vi "CursorDraw.vi"(8 "error in (no error)":errorcluster, 9 "Coords":T1, 11 "Gviewer in":refnum<class "Gviewer.lvclass">) -> (0 "error out":errorcluster, 3 "Gviewer out":refnum<class "Gviewer.lvclass">)   [LabVIEW 2020, in "Sgraph_lib_V1.lvlib" / "Gviewer.lvclass"]
doc: "Draw info at cursor point"
uses:
  Gviewer.lvclass
  <vilib>/Utility/miscctls.llb/LVPoint32TypeDef.ctl
  Gviewer.lvclass/Gviewer.ctl
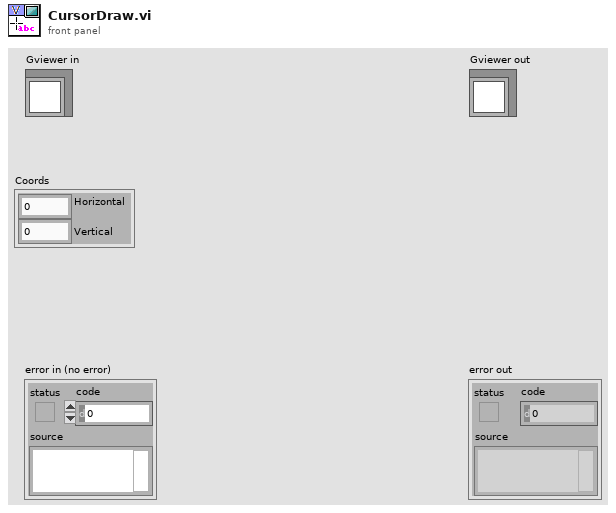
[diagram p1: front panel]
types:
  T1 = typedef "LVPoint32TypeDef.ctl" = cluster{"Horizontal":i32, "Vertical":i32}
  T2 = cluster{"horizontal":enum16{"left", "center", "right"}, "vertical":enum16{"top", "center", "bottom"}}
  T3 = typedef "LVRectTypeDef.ctl" = cluster{"Left":i16, "Top":i16, "Right":i16, "Bottom":i16}
  T4 = typedef "Sgraph_lib_V1.lvlib/Gviewer.lvclass/Typedef_Live.ctl" = enum16{"Live View", "Freeze"}
  T5 = typedef "Sgraph_lib_V1.lvlib/FAMM.lvclass/FAMM_reply_datagram.ctl" = cluster{"GraphName":string, "Time-Start":timestamp, "Time-End":timestamp, "TimeSpan":dbl, "Live":T4, "WAQ_section":T6, "EAQ_section":T7, "PAQ_section":T8, "Layer":i32}
  T6 = typedef "Sgraph_lib_V1.lvlib/FAMM.lvclass/FAMM_reply_WAQdata.ctl" = cluster{"Boolean":bool}
  T7 = typedef "Sgraph_lib_V1.lvlib/FAMM.lvclass/FAMM_reply_EAQdata.ctl" = cluster{"Boolean":bool}
  T8 = typedef "Sgraph_lib_V1.lvlib/FAMM.lvclass/FAMM_reply_PAQdata.ctl" = cluster{"Tags":string[], "time stamp":timestamp[], "DataSection":cluster{"data":dbl[], "max":dbl[], "min":dbl[], "Status":u32[]}[]}
  T9 = typedef "Sgraph_lib_V1.lvlib/Gviewer.lvclass/LegendSet.ctl" = cluster{"Position":T10, "Size":T11, "Rows":u32, "Select":i32, "Visible":bool}
  T10 = typedef "LVPositionTypeDef.ctl" = cluster{"Left":i32, "Top":i32}
  T11 = typedef "LVBoundsTypeDef.ctl" = cluster{"Width":u32, "Height":u32}
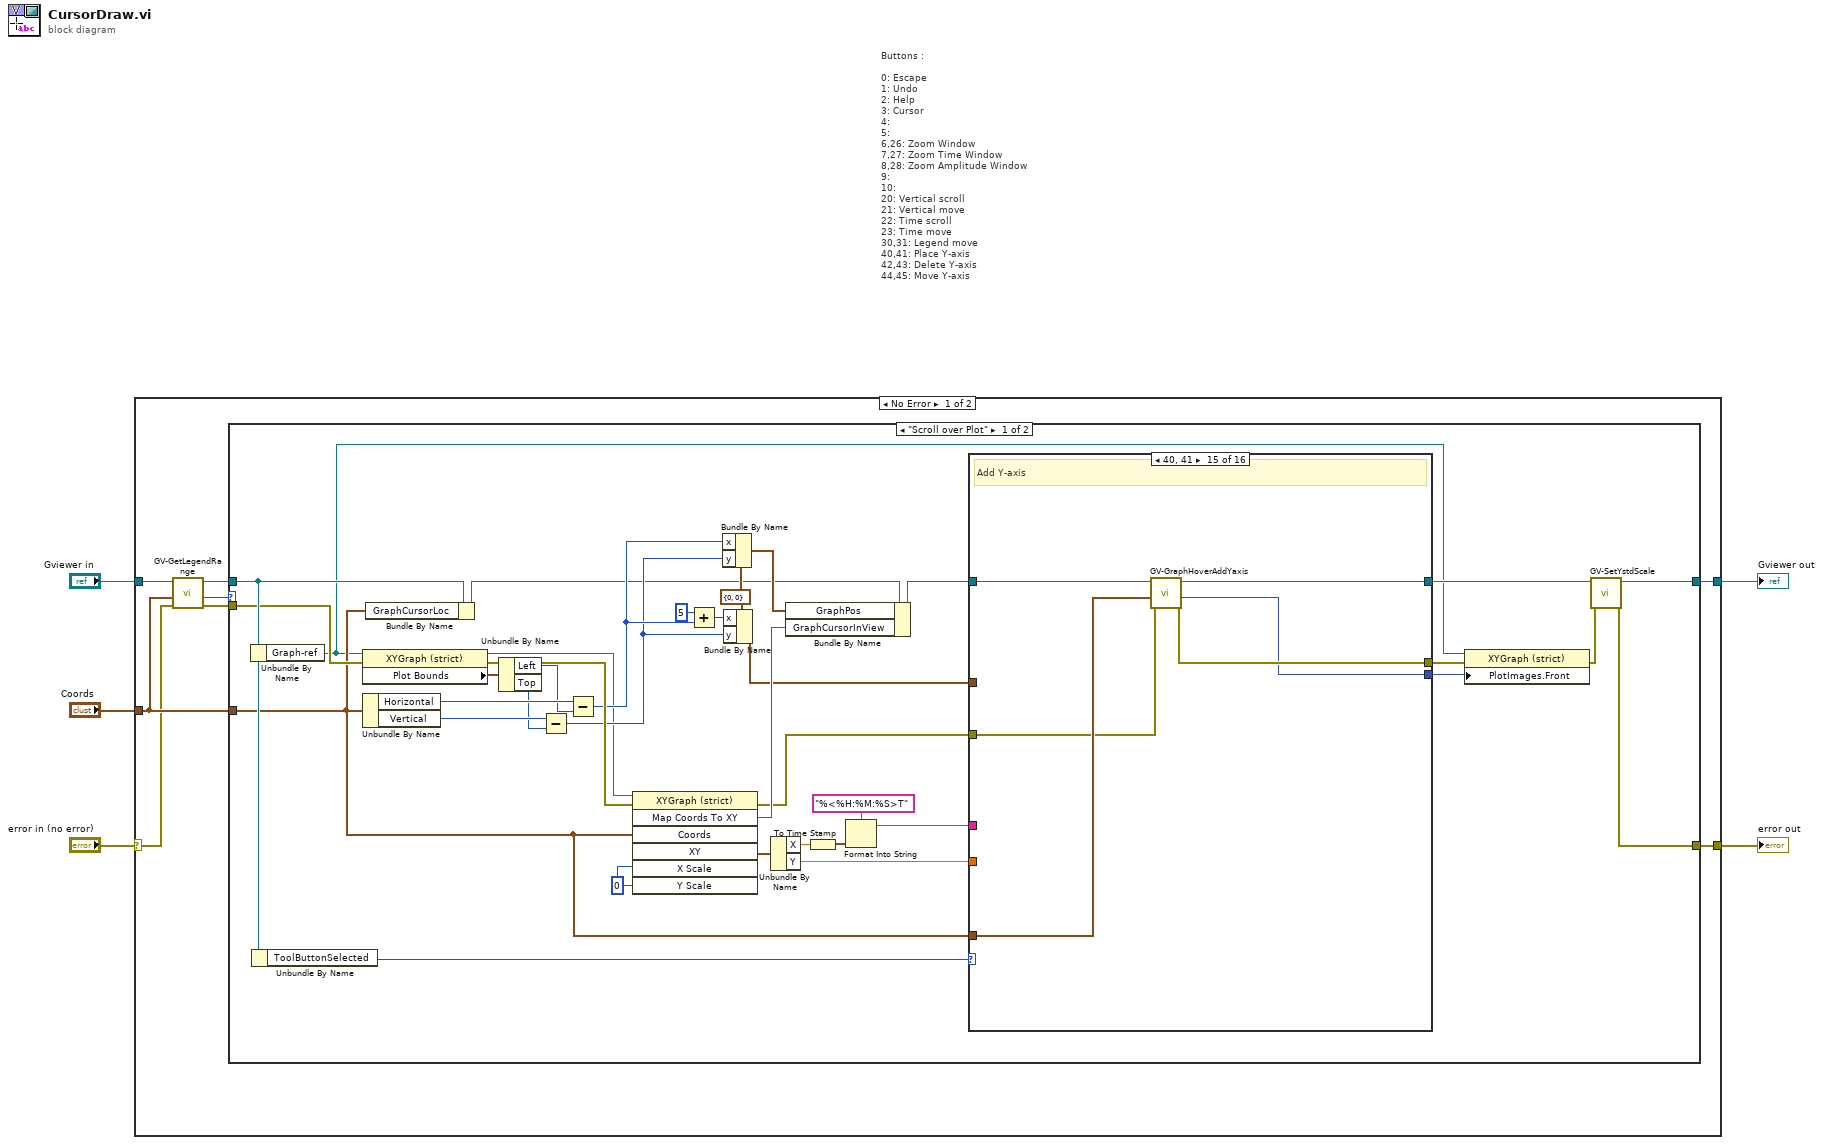
[diagram p0: block diagram]
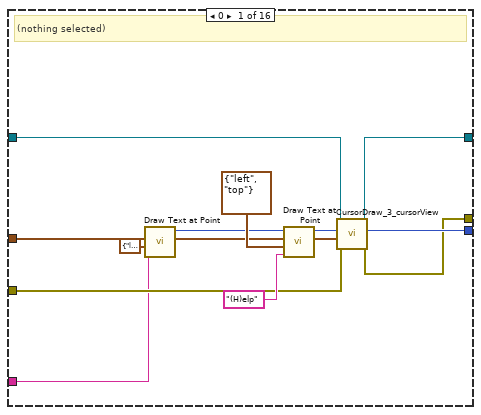
[diagram p2: hidden frame]
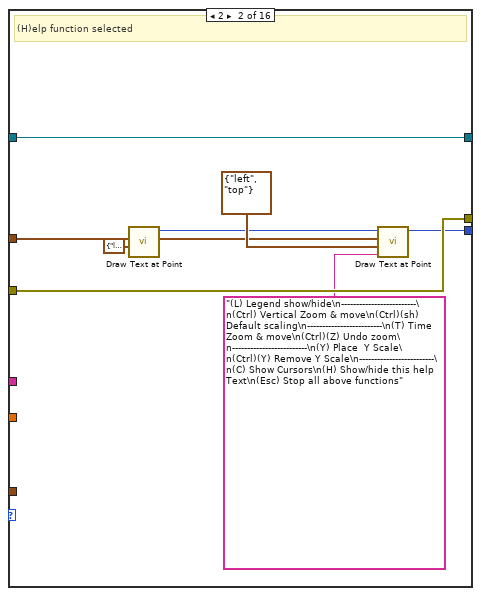
[diagram p3: hidden frame]
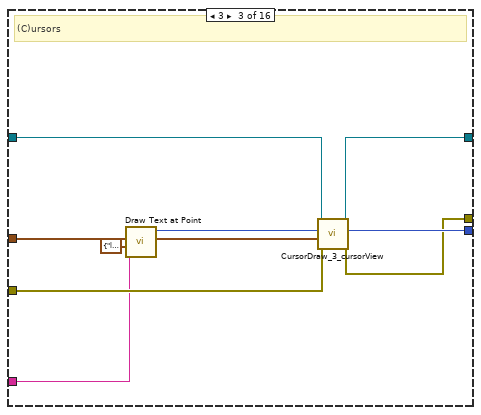
[diagram p4: hidden frame]
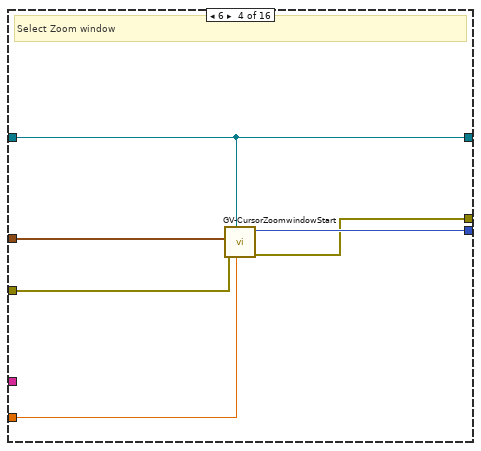
[diagram p5: hidden frame]
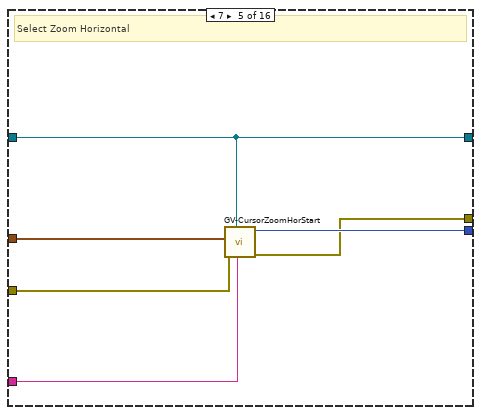
[diagram p6: hidden frame]
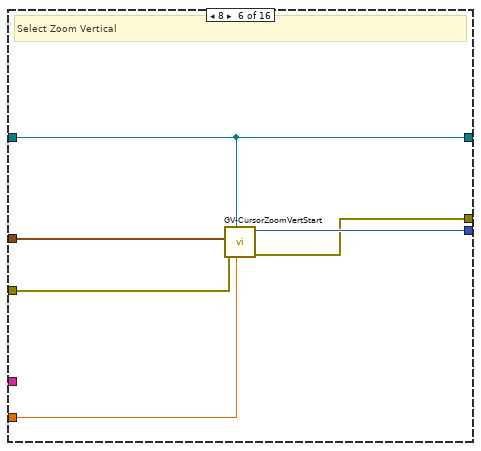
[diagram p7: hidden frame]
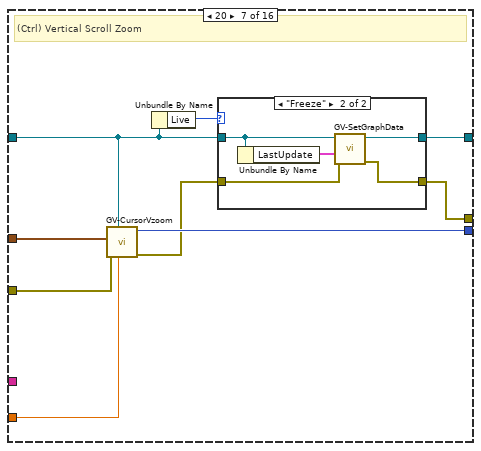
[diagram p8: hidden frame]
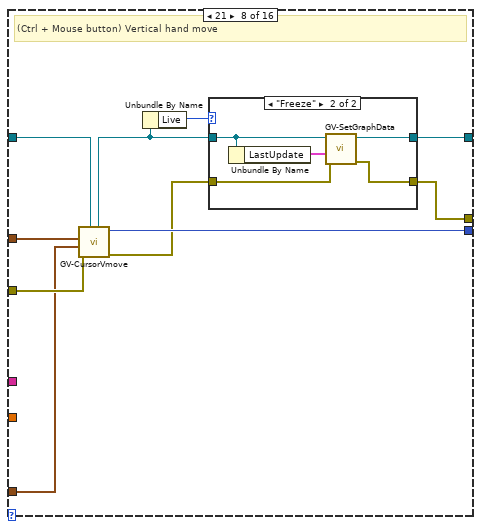
[diagram p10: hidden frame]
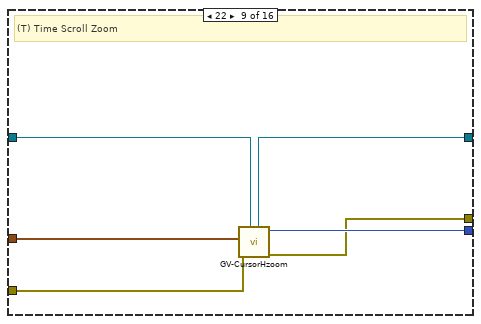
[diagram p12: hidden frame]
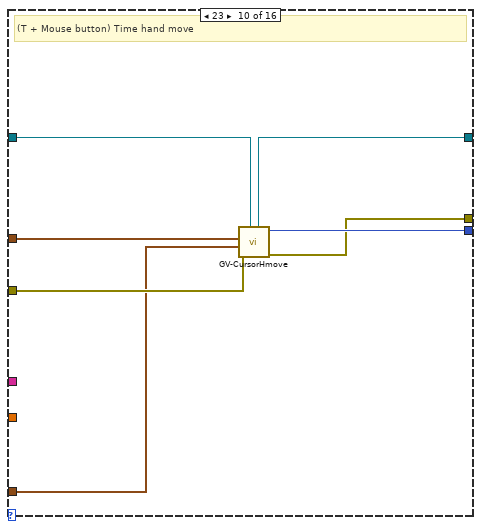
[diagram p13: hidden frame]
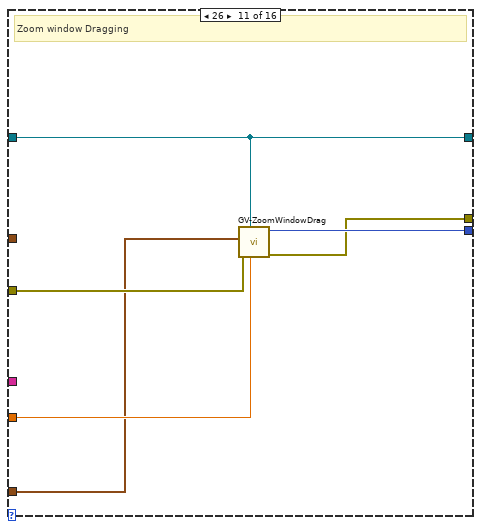
[diagram p14: hidden frame]
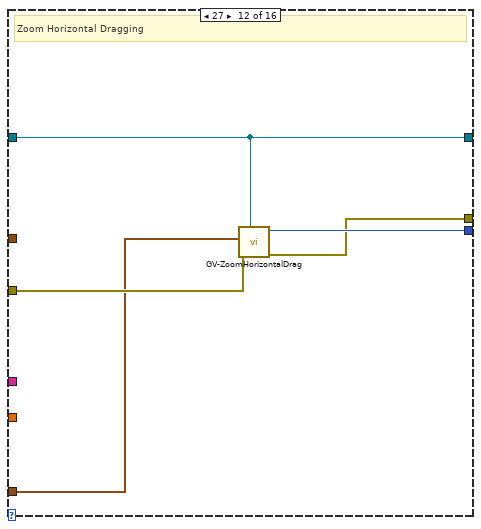
[diagram p15: hidden frame]
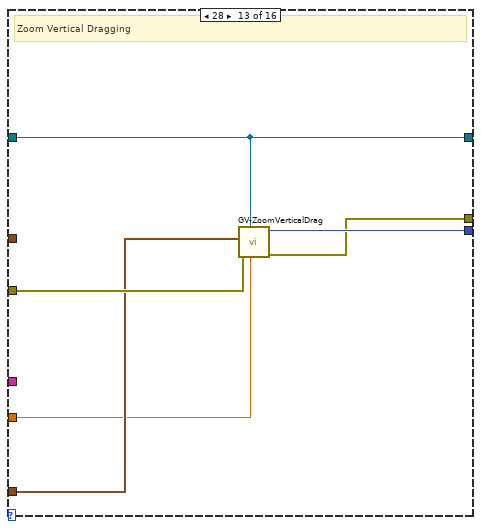
[diagram p16: hidden frame]
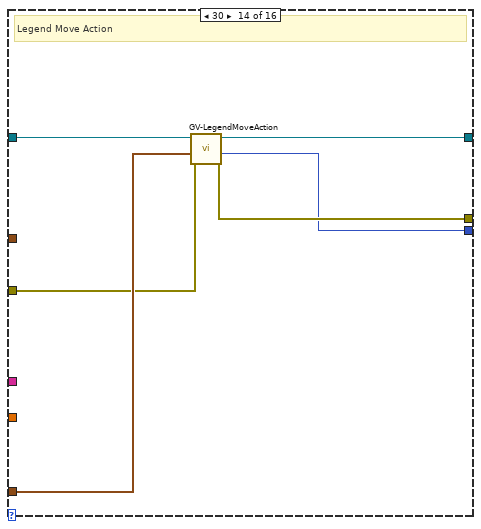
[diagram p17: hidden frame]
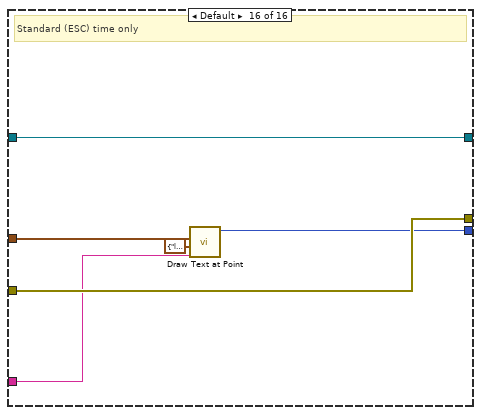
[diagram p18: hidden frame]
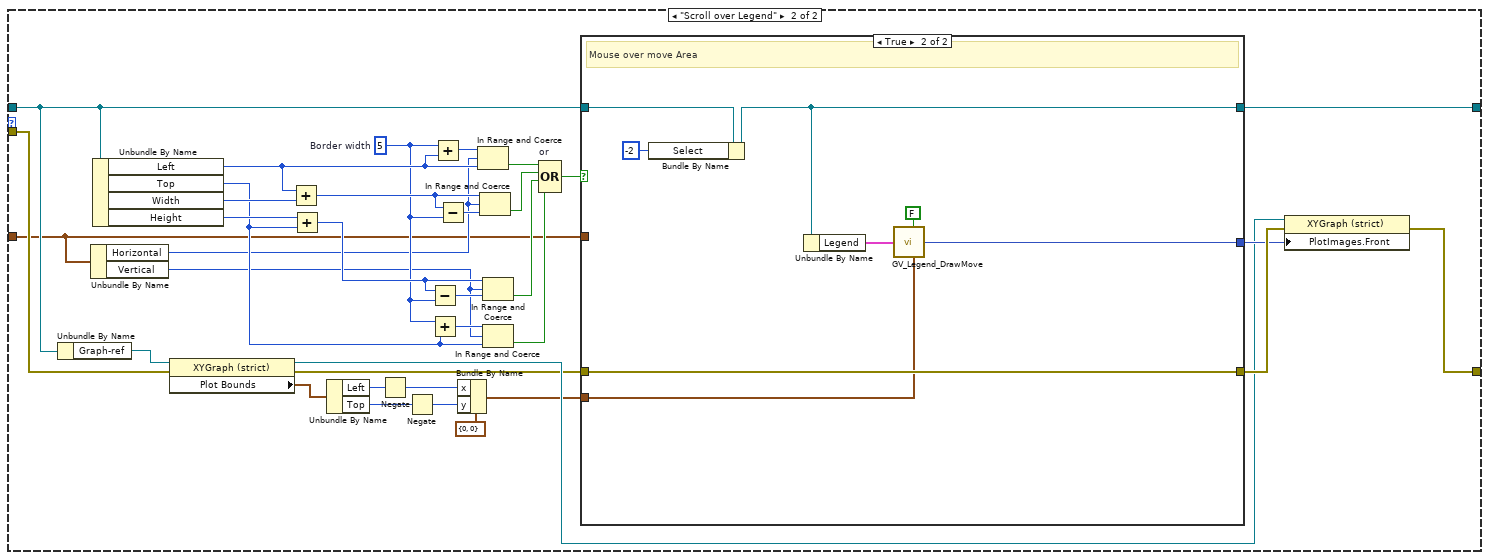
[diagram p19: hidden frame]
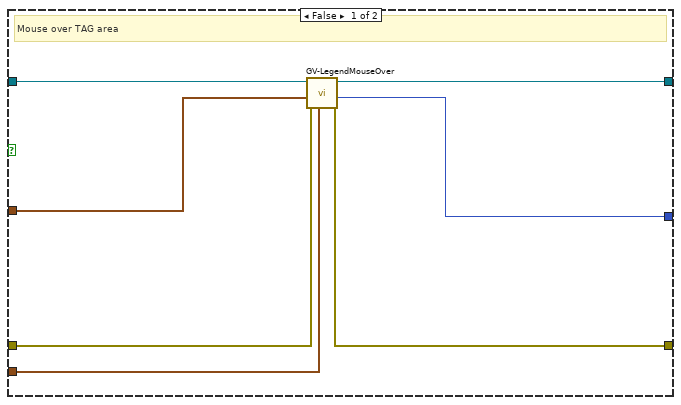
[diagram p20: hidden frame]
diagram:
  # "Buttons :\n\n0: Escape\n1: Undo\n2: Help\n3: Cursor\n4: \n5:\n6,26: Zoom Window\n7,27: Zoom Time Window\n8,28: Zoom Amplitude Window\n9:\n10:\n20: Vertical scroll\n21: Vertical move\n22: Time scroll\n23: Time move\n30,31: Legend move\n40,41: Place Y-axis\n42,43: Delete Y-axis\n44,45: Move Y-axis"
  n1 = case shown="No Error" "error in (no error)" {
    selector: "error in (no error)" -> [w6 w229]
    tunnel: [w12 w229] -> w4
    tunnel: [w13 w228] -> w2
    tunnel: "Gviewer in" -> [w10 w228]
    tunnel: "Coords" -> [w8 _]
    frame No Error {
      n2 = call "GV-GetLegendRange.vi"("error in (no error)"=w6, "Coords"=w8, "Gviewer in"=w10) -> ("error out"=w9:errorcluster, "Where?"=w7:enum16{"Scroll over Plot", "Scroll over Legend"}, "Gviewer out"=w11:refnum<class "Gviewer.lvclass">)  [unwired: 6 in]
      n3 = case shown="\"Scroll over Plot\"" w7 {
        tunnel: [w22 w178] -> w13
        tunnel: [w20 w179] -> w12
        tunnel: w11 -> [w19 w196]
        tunnel: w9 -> [w18 w181]
        tunnel: w8 -> [w17 w180]
        frame "Scroll over Plot" {
          w43 = 0 ("Y Scale")
          w31 = cluster{"x":i16, "y":i16} {"x"=0, "y"=0} ("origin")
          n4 = Unbundle By Name(w19) -> ("Graph-ref"=w14:refnum<vi>)
          n5 = Unbundle By Name(w19) -> ("ToolButtonSelected"=w26:i32)
          n6 = property class="XYGraph (strict)"(reference=w14, error in=w18) -> (reference out=w15:refnum<vi>, error out=w44:errorcluster, "Plot Bounds"=w49:T3)
          n7 = Unbundle By Name(w17) -> ("Horizontal"=w48:i32, "Vertical"=w47:i32)
          n8 = Bundle By Name(cluster=w19, "GraphCursorLoc"=w17) -> (w27:refnum<class "Gviewer.lvclass">)
          n9 = Unbundle By Name(w49) -> ("Left"=w46:i16, "Top"=w45:i16)
          n10 = Subtract(x=w47, y=w45) -> (x-y=w29:i32)
          n11 = Subtract(x=w48, y=w46) -> (x-y=w30:i32)
          n12 = invoke class="XYGraph (strict)" method="Map Coords To XY"(reference=w15, error in=w44, "Coords"=w17, "X Scale"=w43, "Y Scale"=w43) -> (error out=w33:errorcluster, "Map Coords To XY"=w41:bool, "XY"=w42:cluster{"X":dbl, "Y":dbl})  [unwired: 2 in, 4 out]
          n13 = Add(x=5, y=w30) -> (x+y=w36:i32)
          n14 = Bundle By Name(cluster=w31, "x"=w30, "y"=w29) -> (w28:cluster{"x":i16, "y":i16})
          n15 = Bundle By Name(cluster=w31, "x"=w36, "y"=w29) -> (w24:cluster{"x":i16, "y":i16})
          n16 = Unbundle By Name(w42) -> ("X"=w40:dbl, "Y"=w23:dbl)
          n17 = Bundle By Name(cluster=w27, "GraphPos"=w28, "GraphCursorInView"=w41) -> (w35:refnum<class "Gviewer.lvclass">)
          n18 = To Time Stamp(1:w40) -> (0:w39:timestamp)
          n19 = Format Into String(format string="%<%H:%M:%S>T", w39) -> (resulting string=w25:string)  [unwired: 2 in, 1 out]
          n20 = case shown="40, 41" w26 {
            tunnel: w35 -> [w56 w69 w77 w80 w86 w92 w98 w120 w130 w136 w145 w150 w156 w165 w171 w177]
            tunnel: [w58 w67 w76 w84 w90 w96 w105 w118 w135 w142 w148 w153 w159 w160 w166 w174] -> w34
            tunnel: [w57 w69 w78 w80 w86 w92 w101 w115 w131 w137 w145 w150 w156 w163 w169 w177] -> w16
            tunnel: w33 -> [w54 w68 w74 w83 w89 w95 w104 w122 w133 w140 w146 w151 w157 w162 w168 w176]
            tunnel: [w55 w68 w75 w82 w88 w94 w99 w113 w134 w141 w147 w152 w158 w161 w167 w176] -> w32
            tunnel: w25 -> [w50 _ w70 _ w85 _ _ _ _ _ _ _ _ _ _ w173]
            tunnel: w24 -> [w51 w62 w72 w81 w87 w93 w103 w119 w132 w139 _ _ _ _ _ w172]
            tunnel: w23 -> [_ _ _ w79 _ w91 w102 _ _ _ w144 _ w154 _ _ _]
            tunnel: w17 -> [_ _ _ _ _ _ _ w121 _ w138 w143 w149 w155 w164 w170 _]
            frame 0 {
              # "(nothing selected)"
              n21 = call <vilib>:"Draw Text at Point.vi"("text"=w50, "alignment(left, top)"=T2 {"horizontal"=enum."left", "vertical"=enum."bottom"}, "origin"=w51) -> ("new picture"=w52:picture)  [unwired: 7 in, 1 out]
              n22 = call <vilib>:"Draw Text at Point.vi"("text"="(H)elp", "alignment(left, top)"=T2 {"horizontal"=enum."left", "vertical"=enum."top"}, "origin"=w51, "picture"=w52) -> ("new picture"=w59:picture)  [unwired: 6 in, 1 out]
              n23 = call "CursorDraw_3_cursorView.vi"("error in (no error)"=w54, "Pos"=w51, "pict in"=w59, "Gviewer in"=w56) -> ("error out"=w55:errorcluster, "pict out"=w58:picture, "Gviewer out"=w57:refnum<class "Gviewer.lvclass">)  [unwired: 5 in]
            }
            frame 2 {
              # "(H)elp function selected"
              n24 = call <vilib>:"Draw Text at Point.vi"("alignment(left, top)"=T2 {"horizontal"=enum."left", "vertical"=enum."bottom"}, "origin"=w62) -> ("new picture"=w63:picture)  [unwired: 8 in, 1 out]
              n25 = call <vilib>:"Draw Text at Point.vi"("text"="(L) Legend show/hide\n-------------------------\n(Ctrl) Vertical Zoom & move\n(Ctrl)(sh) Default scaling\n-------------------------\n(T) Time Zoom & move\n(Ctrl)(Z) Undo zoom\n-------------------------\n(Y) Place  Y Scale\n(Ctrl)(Y) Remove Y Scale\n-------------------------\n(C) Show Cursors\n(H) Show/hide this help Text\n(Esc) Stop all above functions", "alignment(left, top)"=T2 {"horizontal"=enum."left", "vertical"=enum."top"}, "origin"=w62, "picture"=w63) -> ("new picture"=w67:picture)  [unwired: 6 in, 1 out]
            }
            frame 3 {
              # "(C)ursors"
              n26 = call <vilib>:"Draw Text at Point.vi"("text"=w70, "alignment(left, top)"=T2 {"horizontal"=enum."left", "vertical"=enum."bottom"}, "origin"=w72) -> ("new picture"=w71:picture)  [unwired: 7 in, 1 out]
              n27 = call "CursorDraw_3_cursorView.vi"("error in (no error)"=w74, "Pos"=w72, "pict in"=w71, "Gviewer in"=w77) -> ("error out"=w75:errorcluster, "pict out"=w76:picture, "Gviewer out"=w78:refnum<class "Gviewer.lvclass">)  [unwired: 5 in]
            }
            frame 6 {
              # "Select Zoom window"
              n28 = call "GV-CursorZoomwindowStart.vi"("Y"=w79, "Gviewer in"=w80, "error in (no error)"=w83, "Pos"=w81) -> ("error out"=w82:errorcluster, "pict out"=w84:picture)  [unwired: 6 in]
            }
            frame 7 {
              # "Select Zoom Horizontal"
              n29 = call "GV-CursorZoomHorStart.vi"("time"=w85, "Gviewer in"=w86, "error in (no error)"=w89, "Pos"=w87) -> ("error out"=w88:errorcluster, "pict out"=w90:picture)  [unwired: 6 in]
            }
            frame 8 {
              # "Select Zoom Vertical"
              n30 = call "GV-CursorZoomVertStart.vi"("Y"=w91, "Gviewer in"=w92, "error in (no error)"=w95, "Pos"=w93) -> ("error out"=w94:errorcluster, "pict out"=w96:picture)  [unwired: 6 in]
            }
            frame 20 {
              # "(Ctrl) Vertical Scroll Zoom"
              n31 = call "GV-CursorVzoom.vi"("Y"=w102, "Gviewer in"=w98, "error in (no error)"=w104, "Pos"=w103) -> ("error out"=w100:errorcluster, "pict out"=w105:picture)  [unwired: 6 in]
              n32 = Unbundle By Name(w98) -> ("Live"=w97:T4)
              n33 = case shown="\"Freeze\"" w97 {
                tunnel: [w107 w111] -> w101
                tunnel: w98 -> [w107 w110]
                tunnel: w100 -> [w106 w109]
                tunnel: [w106 w108] -> w99
                frame "Live View", Default {
                }
                frame "Freeze" {
                  n34 = Unbundle By Name(w110) -> ("LastUpdate"=w112:T5)
                  n35 = call "GV-SetGraphData.vi"("error in (no error)"=w109, "GviewerUpdate"=w112, "Gviewer in"=w110) -> ("error out"=w108:errorcluster, "Gviewer out"=w111:refnum<class "Gviewer.lvclass">)  [unwired: 7 in]
                }
              }
            }
            frame 21 {
              # "(Ctrl + Mouse button) Vertical hand move"
              n36 = call "GV-CursorVmove.vi"("Gviewer in"=w120, "error in (no error)"=w122, "New coordinate"=w121, "Pos"=w119) -> ("error out"=w114:errorcluster, "pict out"=w118:picture, "Gviewer out"=w116:refnum<class "Gviewer.lvclass">)  [unwired: 5 in]
              n37 = Unbundle By Name(w116) -> ("Live"=w117:T4)
              n38 = case shown="\"Freeze\"" w117 {
                tunnel: [w124 w128] -> w115
                tunnel: w116 -> [w124 w127]
                tunnel: w114 -> [w123 w126]
                tunnel: [w123 w125] -> w113
                frame "Live View", Default {
                }
                frame "Freeze" {
                  n39 = Unbundle By Name(w127) -> ("LastUpdate"=w129:T5)
                  n40 = call "GV-SetGraphData.vi"("error in (no error)"=w126, "GviewerUpdate"=w129, "Gviewer in"=w127) -> ("error out"=w125:errorcluster, "Gviewer out"=w128:refnum<class "Gviewer.lvclass">)  [unwired: 7 in]
                }
              }
            }
            frame 22 {
              # "(T) Time Scroll Zoom"
              n41 = call "GV-CursorHzoom.vi"("Gviewer in"=w130, "error in (no error)"=w133, "Pos"=w132) -> ("error out"=w134:errorcluster, "pict out"=w135:picture, "Gviewer out"=w131:refnum<class "Gviewer.lvclass">)  [unwired: 6 in]
            }
            frame 23 {
              # "(T + Mouse button) Time hand move"
              n42 = call "GV-CursorHmove.vi"("Gviewer in"=w136, "error in (no error)"=w140, "New coordinate"=w138, "Pos"=w139) -> ("error out"=w141:errorcluster, "pict out"=w142:picture, "Gviewer out"=w137:refnum<class "Gviewer.lvclass">)  [unwired: 5 in]
            }
            frame 26 {
              # "Zoom window Dragging"
              n43 = call "GV-ZoomWindowDrag.vi"("Y"=w144, "Gviewer in"=w145, "error in (no error)"=w146, "Coords"=w143) -> ("error out"=w147:errorcluster, "pict out"=w148:picture)  [unwired: 6 in]
            }
            frame 27 {
              # "Zoom Horizontal Dragging"
              n44 = call "GV-ZoomHorizontalDrag.vi"("Gviewer in"=w150, "error in (no error)"=w151, "Coords"=w149) -> ("error out"=w152:errorcluster, "pict out"=w153:picture)  [unwired: 7 in]
            }
            frame 28 {
              # "Zoom Vertical Dragging"
              n45 = call "GV-ZoomVerticalDrag.vi"("Y"=w154, "Gviewer in"=w156, "error in (no error)"=w157, "Coords"=w155) -> ("error out"=w158:errorcluster, "pict out"=w159:picture)  [unwired: 6 in]
            }
            frame 30 {
              # "Legend Move Action"
              n46 = call "GV-LegendMoveAction.vi"("error in (no error)"=w162, "Coords"=w164, "Gviewer in"=w165) -> ("error out"=w161:errorcluster, "Plot Images:Front"=w160:picture, "Gviewer out"=w163:refnum<class "Gviewer.lvclass">)  [unwired: 6 in]
            }
            frame 40, 41 {
              # "Add Y-axis"
              n47 = call "GV-GraphHoverAddYaxis.vi"("error in (no error)"=w168, "Coords"=w170, "Gviewer in"=w171) -> ("error out"=w167:errorcluster, "Plot Images:Front"=w166:picture, "Gviewer out"=w169:refnum<class "Gviewer.lvclass">)  [unwired: 6 in]
            }
            frame Default {
              # "Standard (ESC) time only"
              n48 = call <vilib>:"Draw Text at Point.vi"("text"=w173, "alignment(left, top)"=T2 {"horizontal"=enum."left", "vertical"=enum."bottom"}, "origin"=w172) -> ("new picture"=w174:picture)  [unwired: 7 in, 1 out]
            }
          }
          n49 = property class="XYGraph (strict)"(reference=w14, error in=w32, "PlotImages.Front"=w34) -> (error out=w21:errorcluster)  [unwired: 1 out]
          n50 = call "GV-SetYstdScale.vi"("error in (no error)"=w21, "Gviewer in"=w16) -> ("error out"=w20:errorcluster, "Gviewer out"=w22:refnum<class "Gviewer.lvclass">)  [unwired: 8 in]
        }
        frame "Scroll over Legend" {
          w204 = 5  # Border width
          n51 = Unbundle By Name(w196) -> ("Graph-ref"=w193:refnum<vi>)
          n52 = Unbundle By Name(w180) -> ("Horizontal"=w191:i32, "Vertical"=w190:i32)
          n53 = Unbundle By Name(w196) -> ("Left"=w211:i32, "Top"=w203:i32, "Width"=w210:u32, "Height"=w207:u32)
          n54 = property class="XYGraph (strict)"(reference=w193, error in=w181) -> (reference out=w188:refnum<vi>, error out=w182:errorcluster, "Plot Bounds"=w192:T3)
          n55 = Add(x=w211, y=w210) -> (x+y=w209:u32)
          n56 = Add(x=w207, y=w203) -> (x+y=w206:u32)
          n57 = Unbundle By Name(w192) -> ("Left"=w186:i16, "Top"=w184:i16)
          n58 = Negate(x=w186) -> (-x=w185:i16)
          n59 = Negate(x=w184) -> (-x=w183:i16)
          n60 = Subtract(x=w206, y=w204) -> (x-y=w205:u32)
          n61 = Add(x=w204, y=w203) -> (x+y=w202:i32)
          n62 = Add(x=w204, y=w211) -> (x+y=w212:i32)
          n63 = Subtract(x=w209, y=w204) -> (x-y=w208:u32)
          n64 = Bundle By Name(cluster=cluster{"x":i16, "y":i16} {"x"=0, "y"=0}, "x"=w185, "y"=w183) -> (w187:cluster{"x":i16, "y":i16})
          n65 = In Range and Coerce(upper limit=w212, x=w191, lower limit=w211) -> (In Range?=w201:bool)  [unwired: 1 out]
          n66 = In Range and Coerce(upper limit=w209, x=w191, lower limit=w208) -> (In Range?=w198:bool)  [unwired: 1 out]
          n67 = In Range and Coerce(upper limit=w206, x=w190, lower limit=w205) -> (In Range?=w199:bool)  [unwired: 1 out]
          n68 = In Range and Coerce(upper limit=w202, x=w190, lower limit=w203) -> (In Range?=w200:bool)  [unwired: 1 out]
          n69 = Compound Arithmetic op=OR "or"(w201, w198, w199, w200) -> (w197:bool)
          n70 = case shown="True" w197 {
            tunnel: w196 -> [w219 w221]
            tunnel: w182 -> [w217 w227]
            tunnel: [w218 w222] -> w178
            tunnel: [w216 w227] -> w195
            tunnel: [w214 w225] -> w194
            tunnel: w187 -> [w213 w224]
            tunnel: w180 -> [w215 _]
            frame False {
              # "Mouse over TAG area"
              n71 = call "GV-LegendMouseOver.vi"("Origin"=w213, "error in (no error)"=w217, "Coords"=w215, "Gviewer in"=w219) -> ("error out"=w216:errorcluster, "image"=w214:picture, "Gviewer out"=w218:refnum<class "Gviewer.lvclass">)  [unwired: 5 in]
            }
            frame True {
              # "Mouse over move Area"
              n72 = Bundle By Name(cluster=w221, "Select"=-2 ("Legend.Select")) -> (w222:refnum<class "Gviewer.lvclass">)
              n73 = Unbundle By Name(w222) -> ("Legend"=w226:T9)
              n74 = call "GV_Legend_DrawMove.vi"("Legend"=w226, "Select"=FALSE, "Origin"=w224) -> ("Image"=w225:picture)  [unwired: 6 in]
            }
          }
          n75 = property class="XYGraph (strict)"(reference=w188, error in=w195, "PlotImages.Front"=w194) -> (error out=w179:errorcluster)  [unwired: 1 out]
        }
      }
    }
    frame Error {
    }
  }
  "error out" <- w4
  "Gviewer out" <- w2
